vi "user initialization.vi"(8 "error in":errorcluster, 10 "configuration in":refnum<class "control module configuration.lvclass">, 11 "fixed channel runtime in":refnum<class "MotionModule runtime.lvclass">) -> (0 "error out":errorcluster, 3 "fixed channel runtime out":refnum<class "MotionModule runtime.lvclass">)   [LabVIEW 2017, in "MotionModule runtime.lvclass"]
uses:
  MotionModule runtime.lvclass
  <vilib>/NI/DCAF/Tag Editor Core/control module/configuration/control module configuration.lvclass
  configuration/MotionModule configuration.lvclass
  SoftmotionClass/SoftmotionAxis/SoftmotionAxis.lvclass
  <vilib>/NI/DCAF/Tag Editor Core/control module/runtime/control module runtime.lvclass
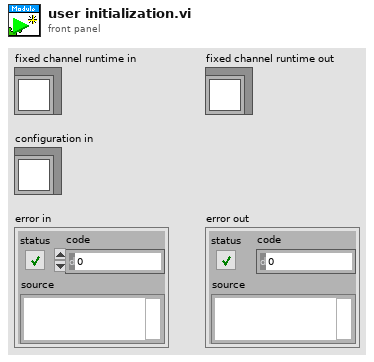
[diagram p1: front panel]
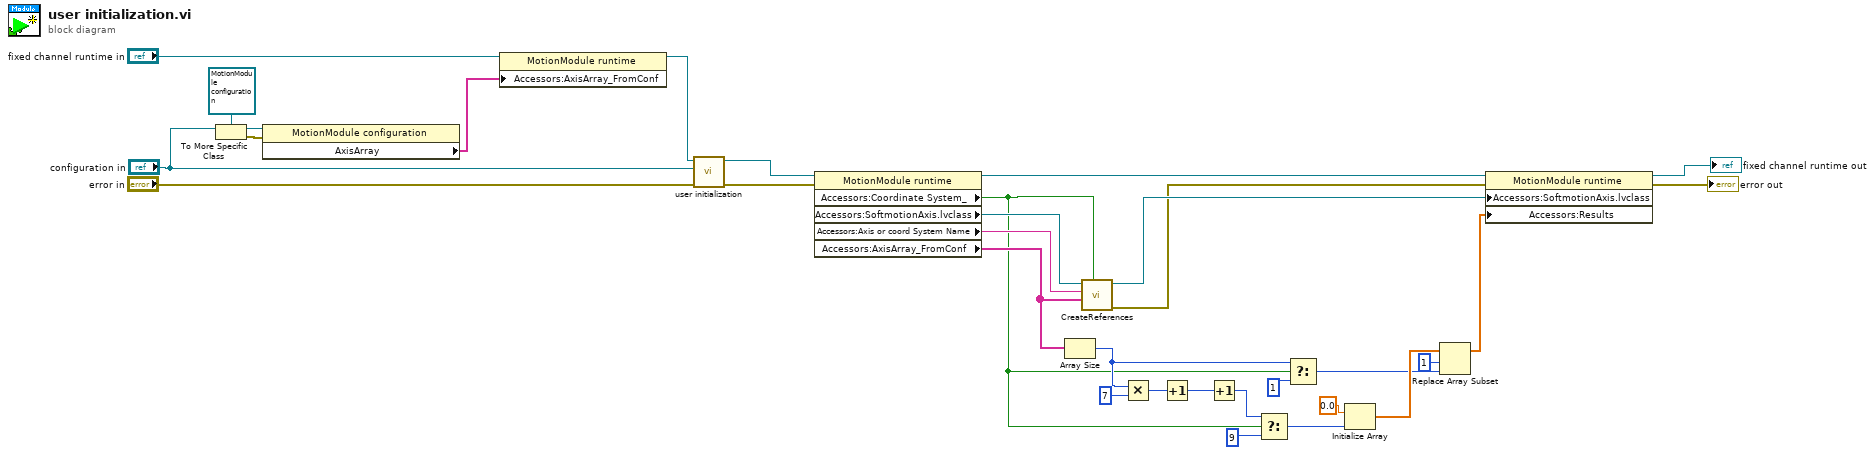
[diagram p0: block diagram]
diagram:
  n1 = To More Specific Class(target class=refnum<class "MotionModule configuration.lvclass"> refnum ("MotionModule configuration"), reference="configuration in") -> (specific class reference=w29:refnum<class "MotionModule configuration.lvclass">, error out=w26:errorcluster)  [unwired: 1 in]
  n2 = property class="MotionModule configuration"(reference=w29, error in=w26) -> ("AxisArray"=w27:string[])  [unwired: 2 out]
  n3 = property class="MotionModule runtime"(reference="fixed channel runtime in", "Accessors:AxisArray_FromConf"=w27) -> (reference out=w31:refnum<class "MotionModule runtime.lvclass">)  [unwired: 1 in, 1 out]
  n4 = call-parent "user initialization.vi"("error in"="error in", "configuration in"="configuration in", "fixed channel runtime in"=w31) -> ("error out"=w20:errorcluster, "fixed channel runtime out"=w21:refnum<class "MotionModule runtime.lvclass">)  [unwired: 7 in]
  n5 = property class="MotionModule runtime"(reference=w21, error in=w20) -> (reference out=w24:refnum<class "MotionModule runtime.lvclass">, "Accessors:Coordinate System_"=w1:bool, "Accessors:SoftmotionAxis.lvclass"=w23:refnum<class "SoftmotionAxis.lvclass">, "Accessors:Axis or coord System Name"=w16:string, "Accessors:AxisArray_FromConf"=w15:string[])  [unwired: 1 out]
  n6 = Array Size(array=w15) -> (size(s)=w4:i32)
  n7 = call-dynamic "CreateReferences.vi"("Coorinate System?"=w1, "AxisArray_FromConf"=w15, "Axis Name"=w16, "SoftmotionAxis in"=w23) -> ("error out"=w17:errorcluster, "SoftmotionAxis out"=w18:refnum<class "SoftmotionAxis.lvclass">)  [unwired: 6 in]
  n8 = Multiply(x=w4, y=7) -> (x*y=w7:i32)
  n9 = Increment(x=w7) -> (x+1=w6:i32)
  n10 = Increment(x=w6) -> (x+1=w13:i32)
  n11 = Select(t=w13, s=w1, f=9) -> (s? t:f=w10:i32)
  n12 = Select(t=w4, s=w1, f=1) -> (s? t:f=w3:i32)
  n13 = Initialize Array(0.0, w10) -> (w9:dbl[])
  n14 = Replace Array Subset(array=w9, new element=w3, index=1) -> (w8:dbl[])
  n15 = property class="MotionModule runtime"(reference=w24, error in=w17, "Accessors:SoftmotionAxis.lvclass"=w18, "Accessors:Results"=w8) -> (reference out=→"fixed channel runtime out":refnum<class "MotionModule runtime.lvclass">, error out=→"error out":errorcluster)
